vi "ZM-HWM-writePrelaunchSettings.vi"(8 "error in (no error)":errorcluster, 10 "settings":T1={"hardware"=refnum, "intervalMs"=500}, 11 "ZM-HWM-hardware_manager in":refnum<class "ZM-HWM-hardware_manager.lvclass">) -> (0 "error out":errorcluster, 3 "ZM-HWM-hardware_manager out":refnum<class "ZM-HWM-hardware_manager.lvclass">)   [LabVIEW 2020, in "ZM-HWM-hardware_manager.lvlib" / "ZM-HWM-hardware_manager.lvclass"]
doc: "Public custom accessor: writes the pre-launch settings. The caller fills ZM-HWM-PRELAUNCH_SETTINGS (hardware object, intervalMs) and then launches the actor."
uses:
  ZM-HWM-hardware_manager.lvclass
  hardware/ZM-HW-hardware/ZM-HW-hardware/ZM-HW-hardware.lvclass
  ZM-HWM-hardware_manager.lvclass/ZM-HWM-hardware_manager.ctl
  ZM-HWM-PRELAUNCH_SETTINGS.ctl
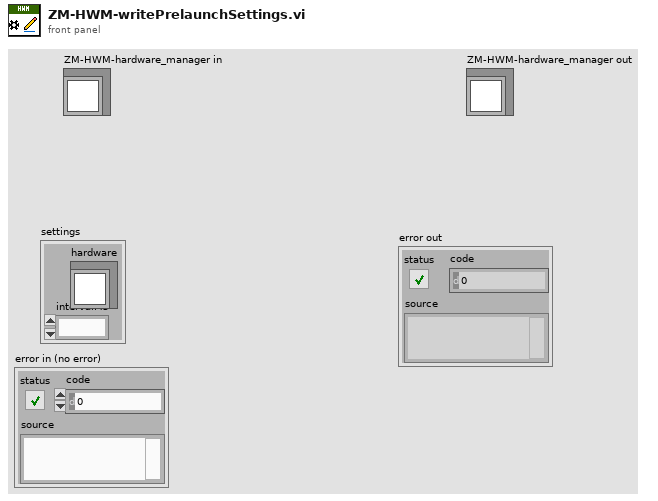
[diagram p1: front panel]
types:
  T1 = typedef "ZM-HWM-hardware_manager.lvlib/ZM-HWM-hardware_manager.lvclass/ZM-HWM-PRELAUNCH_SETTINGS.ctl" = cluster{"hardware":refnum<class "ZM-HW-hardware.lvclass">, "intervalMs":u32}
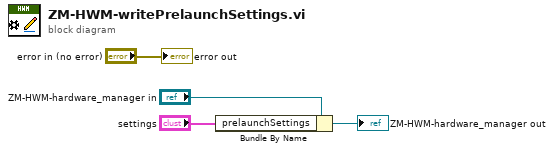
[diagram p0: block diagram]
diagram:
  n1 = Bundle By Name(cluster="ZM-HWM-hardware_manager in", "prelaunchSettings"="settings") -> (→"ZM-HWM-hardware_manager out":refnum<class "ZM-HWM-hardware_manager.lvclass">)
  "error out" <- "error in (no error)"
